vi "DSS-Tests-flatten_dbl_complex.vi"(11 "pair":cluster{"a":dbl[], "b":cdb[]}) -> (3 "flat":dbl[](array[numeric]))   [LabVIEW 2020, in "DSS-Tests.lvlib"]
doc: "Flattens a cluster of a 1D DBL array and a 1D complex DBL array into one 1D DBL array: the DBL array's length and elements, then the complex array's length, real parts and imaginary parts."
uses:
  DSS-Tests.lvlib
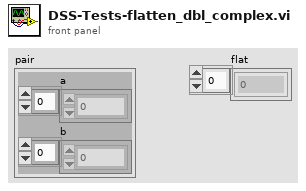
[diagram p1: front panel]
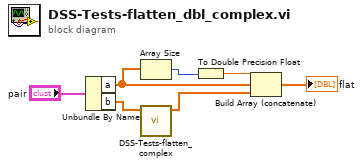
[diagram p0: block diagram]
diagram:
  n1 = Unbundle By Name("pair") -> ("a"=w2:dbl[], "b"=w3:cdb[])
  n2 = Array Size(array=w2) -> (size(s)=w4:i32)
  n3 = call "DSS-Tests-flatten_complex.vi"("values"=w3) -> ("flat"=w6:dbl[])  [unwired: 10 in]
  n4 = To Double Precision Float(number=w4) -> (double precision float=w5:dbl)
  n5 = Build Array (concatenate)(w5, w2, w6) -> (→"flat":dbl[])
